vi "query Swept SA - Trace Values.vi"(8 "error in (no error)":errorcluster, 10 "Trace Index":u32, 11 "FSV-40N in":refnum<class "FSV-40N.lvclass">) -> (0 "error out":errorcluster, 2 "Trace Values":T1 {"Frequency" format="%#_6p"}, 3 "FSV-40N out":refnum<class "FSV-40N.lvclass">)   [LabVIEW 2023, in "Spectrum Analyzer.lvlib" / "FSV-40N.lvclass"]
uses:
  FSV-40N.lvclass
  TYPE DEFINITION/TYPE Trace Value Array.ctl
  FSV-40N.lvclass/FSV-40N.ctl
  Spectrum Analyzer.lvlib
panel:
  out "size(s)":i32
  out "number 3":dbl
  out "number 2":dbl
  out "number":i32
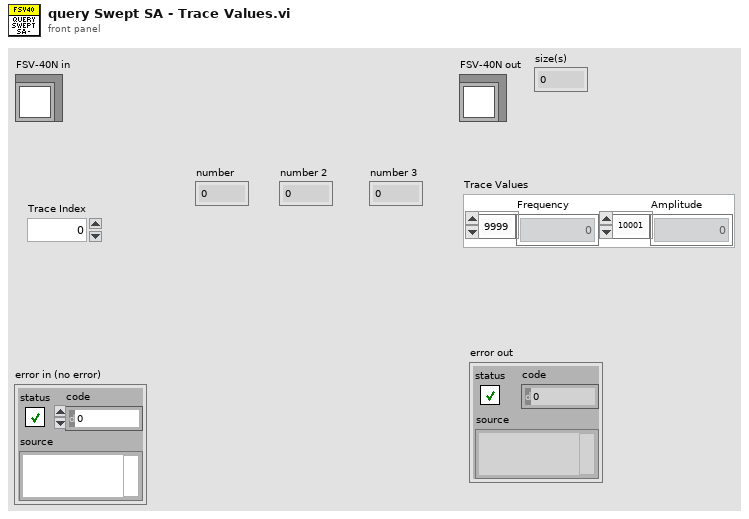
[diagram p1: front panel]
types:
  T1 = typedef "Spectrum Analyzer.lvlib/TYPE Trace Value Array.ctl" = cluster{"Frequency":dbl[], "Amplitude":dbl[]}
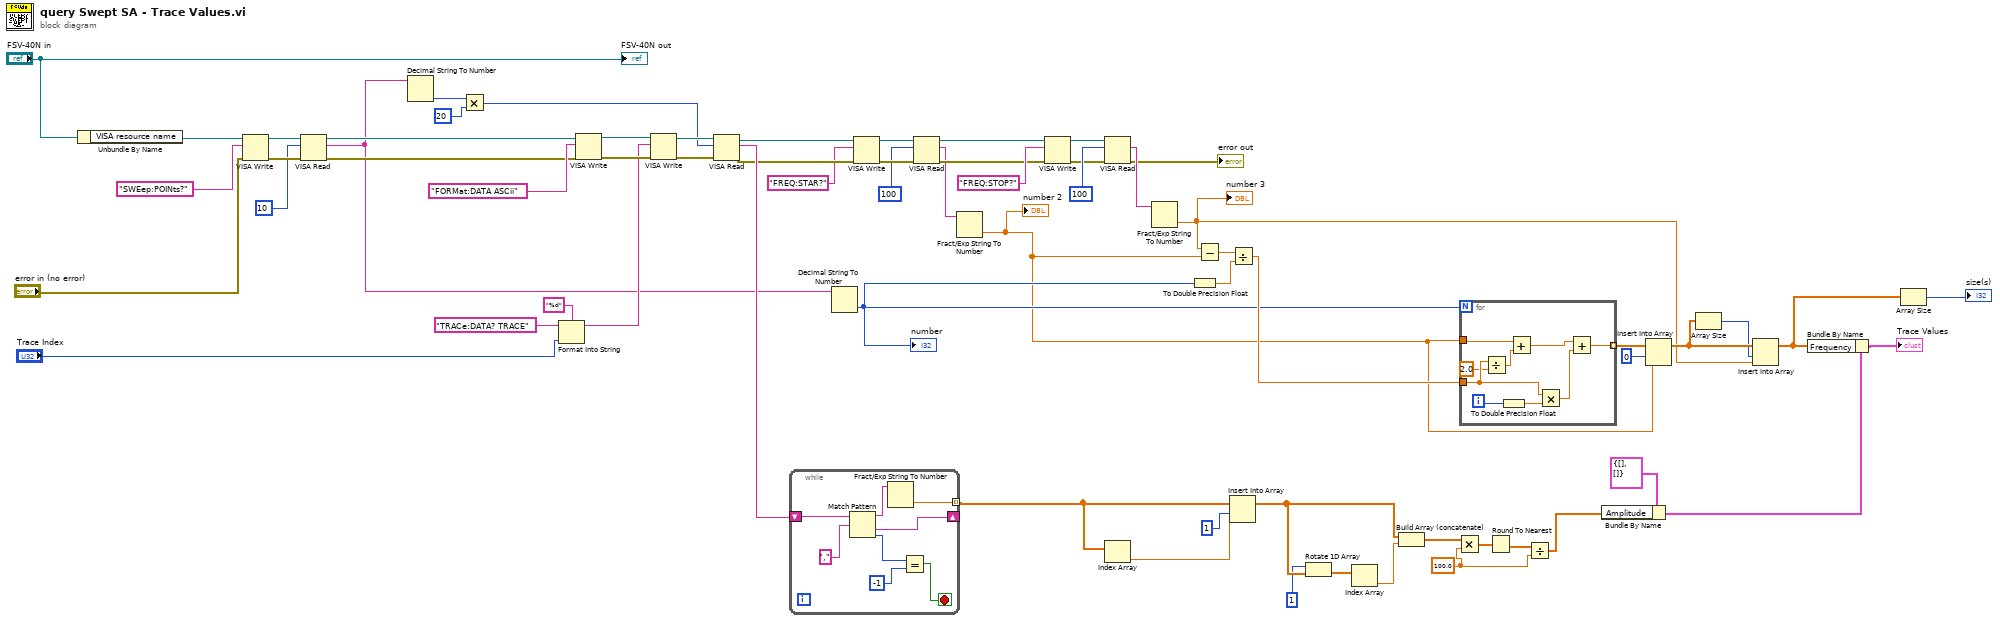
[diagram p0: block diagram]
diagram:
  w7 = 100.0
  n1 = Unbundle By Name("FSV-40N in") -> ("VISA resource name"=w1:refnum<visa-resource-name>)
  n2 = VISA Write(VISA resource name=w1, write buffer="SWEep:POINts?", error in (no error)="error in (no error)") -> (VISA resource name out=w54:refnum<visa-resource-name>, error out=w53:errorcluster)  [unwired: 1 out]
  n3 = VISA Read(VISA resource name=w54, byte count=u32 10, error in (no error)=w53) -> (VISA resource name out=w51:refnum<visa-resource-name>, read buffer=w30:string, error out=w50:errorcluster)  [unwired: 1 out]
  n4 = Decimal String To Number(string=w30) -> (number=w49:i32)  [unwired: 2 in, 1 out]
  n5 = Multiply(x=w49, y=20) -> (x*y=w47:i32)
  n6 = Format Into String(format string="%d", initial string="TRACe:DATA? TRACE" ("write buffer"), "Trace Index") -> (resulting string=w58:string)  [unwired: 1 in, 1 out]
  n7 = VISA Write(VISA resource name=w51, write buffer="FORMat:DATA ASCii", error in (no error)=w50) -> (VISA resource name out=w63:refnum<visa-resource-name>, error out=w62:errorcluster)  [unwired: 1 out]
  n8 = VISA Write(VISA resource name=w63, write buffer=w58, error in (no error)=w62) -> (VISA resource name out=w57:refnum<visa-resource-name>, error out=w56:errorcluster)  [unwired: 1 out]
  n9 = VISA Read(VISA resource name=w57, byte count=w47, error in (no error)=w56) -> (VISA resource name out=w44:refnum<visa-resource-name>, read buffer=w46:string, error out=w43:errorcluster)  [unwired: 1 out]
  n10 = while {
    shift-right: [w68] -> _
    shift-left: w46 -> [w73]
    tunnel: [w66] -> w19 mode=indexing
    stop <- w69 stop-if-true
    n11 = Match Pattern(string=w73, regular expression=",") -> (before substring=w67:string, after substring=w68:string, offset past match=w71:i32)  [unwired: 1 in, 1 out]
    n12 = Fract/Exp String To Number(string=w67) -> (number=w66:dbl)  [unwired: 3 in, 1 out]
    n13 = Equal?(x=w71, y=-1) -> (x = y?=w69:bool)
  }
  n14 = Decimal String To Number(string=w30) -> (number=w22:i32)  [unwired: 2 in, 1 out]
  "number" <- w22
  n15 = VISA Write(VISA resource name=w44, write buffer="FREQ:STAR?", error in (no error)=w43) -> (VISA resource name out=w41:refnum<visa-resource-name>, error out=w40:errorcluster)  [unwired: 1 out]
  n16 = VISA Read(VISA resource name=w41, byte count=u32 100, error in (no error)=w40) -> (VISA resource name out=w34:refnum<visa-resource-name>, read buffer=w32:string, error out=w33:errorcluster)  [unwired: 1 out]
  n17 = Fract/Exp String To Number(string=w32) -> (number=w13:dbl)  [unwired: 3 in, 1 out]
  "number 2" <- w13
  n18 = VISA Write(VISA resource name=w34, write buffer="FREQ:STOP?", error in (no error)=w33) -> (VISA resource name out=w36:refnum<visa-resource-name>, error out=w37:errorcluster)  [unwired: 1 out]
  n19 = VISA Read(VISA resource name=w36, byte count=u32 100, error in (no error)=w37) -> (read buffer=w31:string, error out=→"error out":errorcluster)  [unwired: 2 out]
  n20 = Index Array(array=w19) -> (element=w18:dbl)  [unwired: 1 in]
  n21 = Fract/Exp String To Number(string=w31) -> (number=w4:dbl)  [unwired: 3 in, 1 out]
  "number 3" <- w4
  n22 = To Double Precision Float(number=w22) -> (double precision float=w28:dbl)
  n23 = Subtract(x=w4, y=w13) -> (x-y=w29:dbl)
  n24 = Insert Into Array(array=w19, index=1, new element=w18) -> (w17:dbl[])
  n25 = Divide(x=w29, y=w28) -> (x/y=w27:dbl)
  n26 = Rotate 1D Array(1:w17, 2:1 ("n")) -> (0:w12:dbl[])
  n27 = Index Array(array=w12) -> (element=w11:dbl)  [unwired: 1 in]
  n28 = Build Array (concatenate)(w17, w11) -> (w10:dbl[])
  n29 = Multiply(x=w10, y=w7) -> (x*y=w9:dbl[])
  n30 = for {
    N: w22 -> [_]
    tunnel: w13 -> [w78]
    tunnel: w27 -> [w75]
    tunnel: [w79] -> w15 mode=indexing
    i -> [w82]
    n31 = Divide(x=w75, y=2.0) -> (x/y=w76:dbl)
    n32 = To Double Precision Float(number=w82) -> (double precision float=w81:dbl)
    n33 = Add(x=w78, y=w76) -> (x+y=w77:dbl)
    n34 = Multiply(x=w75, y=w81) -> (x*y=w80:dbl)
    n35 = Add(x=w77, y=w80) -> (x+y=w79:dbl)
  }
  n36 = Round To Nearest(number=w9) -> (nearest integer value=w8:dbl[])
  n37 = Divide(x=w8, y=w7) -> (x/y=w6:dbl[])
  n38 = Bundle By Name(cluster=T1 {"Frequency"=[], "Amplitude"=[]} ("Trace Values 2"), "Amplitude"=w6) -> (w26:T1)
  n39 = Insert Into Array(array=w15, index=0, new element=w13) -> (w5:dbl[])
  n40 = Array Size(array=w5) -> (size(s)=w3:i32)
  n41 = Insert Into Array(array=w5, index=w3, new element=w4) -> (w2:dbl[])
  n42 = Bundle By Name(cluster=w26, "Frequency"=w2) -> (→"Trace Values":T1)
  n43 = Array Size(array=w2) -> (size(s)=→"size(s)":i32)
  "FSV-40N out" <- "FSV-40N in"
